vi "New (Multi Trigger).vi"(6 "file name format (\"logfile_%<%Y-%m-%d_%H-%M-%S>T.log\")":string="logfile_%<%Y-%m-%d_%H-%M-%S>T.log", 7 "cleanup filter (30 days)":refnum<class "CleanupFilter.lvclass">, 8 "error in":errorcluster, 9 "rollover triggers (50 MB)":refnum<class "RolloverTrigger.lvclass">[](array[class]), 10 "formatter (JSON)":refnum<class "Formatter.lvclass">, 11 "log directory (<app dir>/logs)":path) -> (0 "error out":errorcluster, 2 "events":T1, 3 "file handler":refnum<class "File Handler.lvclass">)   [LabVIEW 2018, in "GLog.lvlib" / "File Handler.lvclass"]
uses:
  File Handler.lvclass
  extension/formatter_interface/Formatter.lvclass
  RolloverTrigger/RolloverTrigger.lvclass
  Events.ctl
  File Update Event.ctl
  CleanupFilter/CleanupFilter.lvclass
  RolloverTrigger.Multi/RolloverTrigger.Multi.lvclass
  C:/Users/Colin/Documents/software_projects/labview/glog/src/api/configuration/handlers/file_handler/RolloverTrigger/RolloverTrigger.lvclass
panel:
  # "Connector Pane"
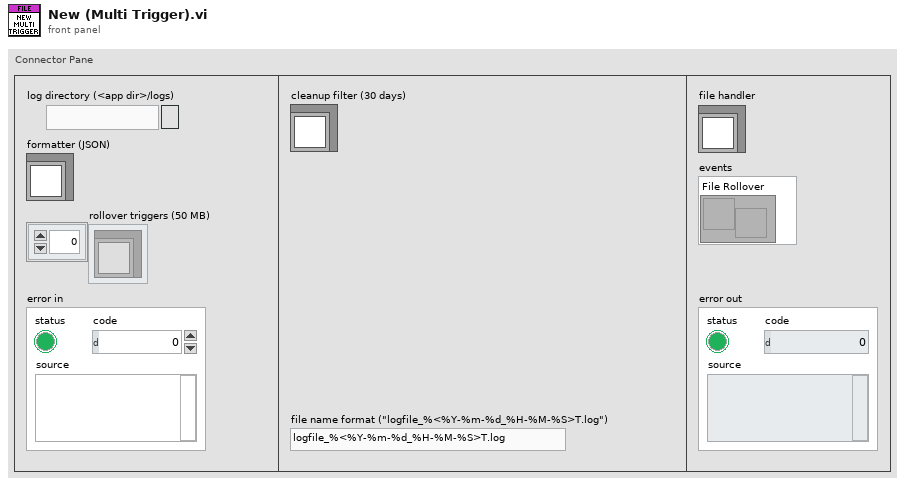
[diagram p1: front panel]
types:
  T1 = typedef "GLog.lvlib/File Handler.lvclass/Events.ctl" = cluster{"File Rollover":refnum<user-event>}
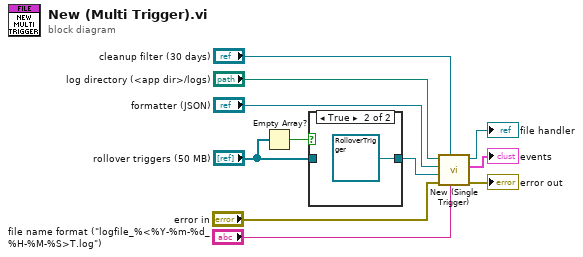
[diagram p0: block diagram]
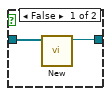
[diagram p2: hidden frame]
diagram:
  n1 = Empty Array?(array="rollover triggers (50 MB)") -> (empty?=w3:bool)
  n2 = case shown="True" w3 {
    tunnel: [w13 refnum<class "RolloverTrigger.lvclass"> refnum ("RolloverTrigger.Multi out")] -> w9
    tunnel: "rollover triggers (50 MB)" -> [w12 _]
    frame False {
      n3 = call "New.vi"("triggers"=w12) -> ("RolloverTrigger.Multi out"=w13:refnum<class "RolloverTrigger.Multi.lvclass">)  [unwired: 10 in]
    }
    frame True {
    }
  }
  n4 = call "New (Single Trigger).vi"("file name format (\"logfile_%<%Y-%m-%d_%H-%M-%S>T.log\")"="file name format (\"logfile_%<%Y-%m-%d_%H-%M-%S>T.log\")", "cleanup filter (never)"="cleanup filter (30 days)", "error in"="error in", "rollover trigger (50 MB)"=w9, "formatter (JSON)"="formatter (JSON)", "log directory (<app dir>/logs)"="log directory (<app dir>/logs)") -> ("error out"=→"error out":errorcluster, "events"=→"events":T1, "file handler"=→"file handler":refnum<class "File Handler.lvclass">)  [unwired: 3 in]
